vi "helper_graph_style.vi"(1 "VI Path":string, 2 "BG Color":string="16777215") -> (0 "matched":string, 3 "classes":string, 4 "code":string, 5 "source":string)   [LabVIEW 2026]
doc: "Find the graph control (GraphChart or WaveformGraph) on a VI's front panel by class name and write its Plot Area BG Color, then save the VI in place. All inputs are strings; BG Color is a LabVIEW color integer as decimal text (R + G*256 + B*65536)."
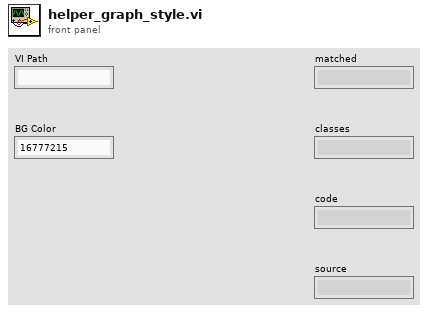
[diagram p1: front panel]
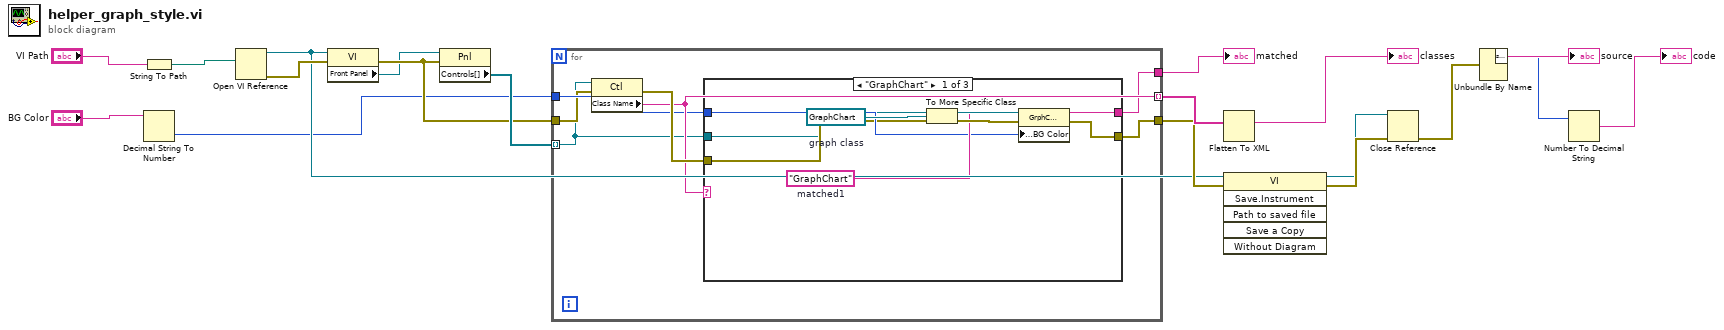
[diagram p0: block diagram]
diagram:
  n1 = String To Path(string="VI Path") -> (path=w3:path)
  n2 = Decimal String To Number(string="BG Color") -> (number=w4:i32)  [unwired: 2 in, 1 out]
  n3 = Open VI Reference(vi path=w3) -> (vi reference=w5:refnum<vi>, error out=w6:errorcluster)  [unwired: 5 in]
  n4 = property class="VI"(reference=w5, error in=w6) -> (error out=w8:errorcluster, "Front Panel"=w7:refnum<vi>)  [unwired: 1 out]
  n5 = property class="Pnl"(reference=w7, error in=w8) -> ("Controls[]"=w9:refnum<vi>[])  [unwired: 2 out]
  n6 = for {
    tunnel: w4 -> [w22]
    tunnel: [w24] -> w11
    tunnel: w8 -> [w21]
    tunnel: w9 -> [w20] mode=indexing
    tunnel: [w25] -> w12 mode=indexing
    tunnel: [w23] -> w10
    n7 = property class="Ctl"(reference=w20, error in=w21) -> (error out=w26:errorcluster, "Class Name"=w25:string)  [unwired: 1 out]
    n8 = case shown="\"b\", Default" w25 {
      tunnel: [w31 w39 w44] -> w24
      tunnel: w22 -> [w29 w37 _]
      tunnel: w20 -> [w27 w35 _]
      tunnel: w26 -> [w28 w36 w43]
      tunnel: [w30 w38 w43] -> w23
      frame "GraphChart" {
        w31 = "GraphChart"  # matched1
        w32 = refnum<vi> refnum  # graph class
        n9 = To More Specific Class(target class=w32, reference=w27, error in=w28) -> (specific class reference=w33:refnum<vi>, error out=w34:errorcluster)
        n10 = property class="GrphChrt"(reference=w33, error in=w34, "Plot Area:Colors:BG Color"=w29) -> (error out=w30:errorcluster)  [unwired: 1 out]
      }
      frame "WaveformGraph" {
        w39 = "WaveformGraph"  # matched2
        w40 = refnum<vi> refnum  # waveform class
        n11 = To More Specific Class(target class=w40, reference=w35, error in=w36) -> (specific class reference=w41:refnum<vi>, error out=w42:errorcluster)
        n12 = property class="GrphChrt"(reference=w41, error in=w42, "Plot Area:Colors:BG Color"=w37) -> (error out=w38:errorcluster)  [unwired: 1 out]
      }
      frame Default {
        w44 = ""  # no match
      }
    }
  }
  "matched" <- w11
  n13 = Flatten To XML(6:w12) -> (2:→"classes":string)
  n14 = invoke class="VI" method="Save.Instrument"(reference=w5, error in=w10) -> (reference out=w13:refnum<vi>, error out=w14:errorcluster)  [unwired: 4 in, 4 out]
  n15 = Close Reference(reference=w13, error in (no error)=w14) -> (error out=w15:errorcluster)
  n16 = Unbundle By Name(w15) -> ("code"=w16:i32, "source"=→"source":string)  [unwired: 1 out]
  n17 = Number To Decimal String(number=w16) -> (decimal integer string=→"code":string)  [unwired: 1 in]
